vi "Get Request Stream.vi"(11 "error in":errorcluster) -> (3 "progressToken":string, 4 "streaming?":bool, 6 "events":refnum<queue>, 8 "cancelled":refnum<queue>, 10 "request id":string, 14 "stream key":string, 15 "error out":errorcluster)   [LabVIEW 2020, in "MCP Server.lvlib"]
doc: "Reads what the tool-side VIs (Report Progress.vi, Cancel Requested.vi) need from the request context of the tools/call that is running: the element of the named queue \"MCP Request Context\", written by Handle MCP Request.vi.\n\nstreaming? is TRUE when the request is answered as a Server-Sent Events stream; then events and cancelled are the two queues of its MCP SSE Response and stream key identifies it. progressToken and request id are the JSON text of params._meta.progressToken and of the request id (null when absent). Outside a request every output is empty or FALSE."
uses:
  MCP Server.lvlib
  7963ba88-334a-429d-a2e7-e93574d76ba4.vi
  c84bf840-9c61-4b0c-85de-9f6fd1d3608d.vi
  <vilib>/JDP Science/JSONtext/Next JSON Value.vi
  <vilib>/JDP Science/JSONtext/String Subset.vi
  <vilib>/JDP Science/JSONtext/Parsing/Advance past next JSON Value (inlined COPY).vi
  <vilib>/JDP Science/JSONtext/Parsing/Advance past whitespace.vi
  <vilib>/JDP Science/JSONtext/Parsing/Advance past String.vi
  <vilib>/JDP Science/JSONtext/Parsing/Advance past Number.vi
  <vilib>/JDP Science/JSONtext/Parsing/Advance past Line Ending.vi
  <vilib>/JDP Science/JSONtext/Parsing/Parse Full Path or Item Name.vi
  <vilib>/JDP Science/JSONtext/Parsing/Advance past Array.vi
  <vilib>/JDP Science/JSONtext/Parsing/Advance past Object.vi
  <vilib>/JDP Science/JSONtext/support/Error Cluster From Code.vi
  <vilib>/JDP Science/JSONtext/Offset/Find Item Locations by Path.vi
  <vilib>/JDP Science/JSONtext/JSON text to Variant.vi
  <vilib>/JDP Science/JSONtext/LVClass Serializer/JSONtext LVClass Serializer.lvclass
  <vilib>/JDP Science/JSONtext/JSONtext.lvlib
panel:
  in  "cancelled type":refnum<queue>
  in  "events type":refnum<queue>
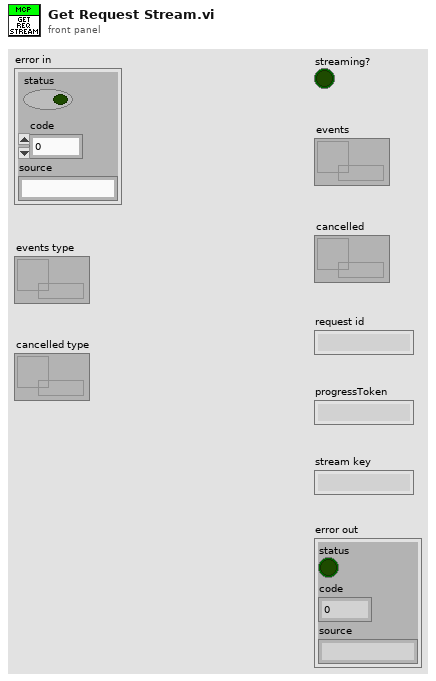
[diagram p1: front panel]
types:
  T1 = typedef "JSONtext.lvlib/JSON Value Type.ctl" = enum16{"Not a JSON Value", "JSON Object", "JSON Array", "String", "Number", "true", "false", "null"}
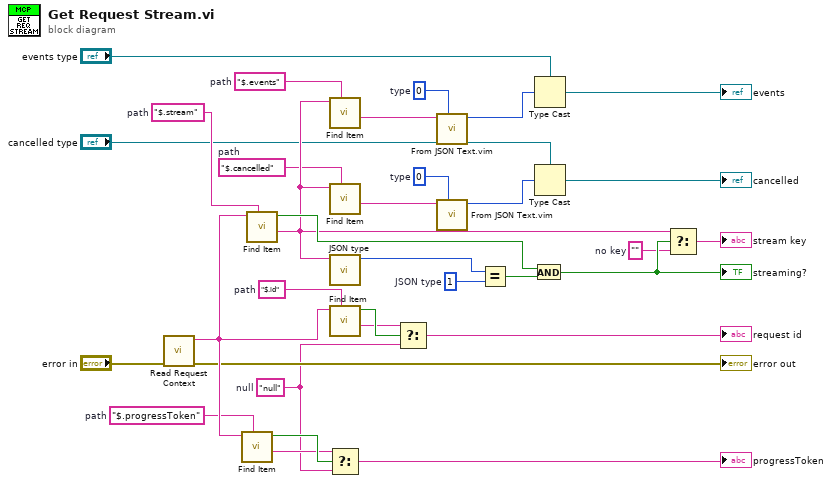
[diagram p0: block diagram]
diagram:
  w13 = ""  # no key
  w12 = "null"  # null
  w11 = "$.id"  # path
  w10 = "$.progressToken"  # path
  w9 = u32 0  # type
  w8 = "$.cancelled"  # path
  w7 = u32 0  # type
  w6 = "$.events"  # path
  w5 = u16 1  # JSON type
  w4 = "$.stream"  # path
  n1 = call "Read Request Context.vi"("error in"="error in") -> ("error out"=→"error out":errorcluster, "context"=w21:string)  [unwired: 8 in, 1 out]
  n2 = call <vilib>:"Find Item.vi"("$Path or Item Name"=w10, "JSON"=w21) -> ("<JSON>"=w24:string, "Found"=w25:bool)  [unwired: 6 in, 2 out]
  n3 = call <vilib>:"Find Item.vi"("$Path or Item Name"=w4, "JSON"=w21) -> ("<JSON>"=w22:string, "Found"=w23:bool)  [unwired: 6 in, 2 out]
  n4 = call <vilib>:"Find Item.vi"("$Path or Item Name"=w6, "JSON"=w22) -> ("<JSON>"=w29:string)  [unwired: 6 in, 3 out]
  n5 = call <vilib>:"Find Item.vi"("$Path or Item Name"=w8, "JSON"=w22) -> ("<JSON>"=w30:string)  [unwired: 6 in, 3 out]
  n6 = call <vilib>:"JSON type.vi"("JSON"=w22) -> ("JSON Value Type"=w28:T1)  [unwired: 9 in, 1 out]
  n7 = call <vilib>:"Find Item.vi"("$Path or Item Name"=w11, "JSON"=w21) -> ("<JSON>"=w26:string, "Found"=w27:bool)  [unwired: 6 in, 2 out]
  n8 = Select(t=w24, s=w25, f=w12) -> (s? t:f=→"progressToken":string)
  n9 = Select(t=w26, s=w27, f=w12) -> (s? t:f=→"request id":string)
  n10 = call "From JSON Text.vim"("Data Type and Default Value"=w7, "JSON"=w29) -> ("Data out"=w32:u32)  [unwired: 8 in, 1 out]
  n11 = call "From JSON Text.vim"("Data Type and Default Value"=w9, "JSON"=w30) -> ("Data out"=w33:u32)  [unwired: 8 in, 1 out]
  n12 = Equal?(x=w28, y=w5) -> (x = y?=w31:bool)
  n13 = And(x=w23, y=w31) -> (x .and. y?=w14:bool)
  "streaming?" <- w14
  n14 = Type Cast(type="events type", x=w32) -> (*(type *) &x=→"events":refnum<queue>)
  n15 = Type Cast(type="cancelled type", x=w33) -> (*(type *) &x=→"cancelled":refnum<queue>)
  n16 = Select(t=w22, s=w14, f=w13) -> (s? t:f=→"stream key":string)
